vi "Generate Tree Data Representation.vi"(8 "error in (no error)":errorcluster, 11 "ParseGDSII in":refnum<class "ParseGDSII.lvclass">) -> (0 "error out":errorcluster, 3 "ParseGDSII out":refnum<class "ParseGDSII.lvclass">)   [LabVIEW 2019, in "ParseGDSII.lvclass"]
uses:
  ParseGDSII.lvclass
  ParseGDSII.lvclass/ParseGDSII.ctl
  Fast Tree/Fast Tree.lvclass
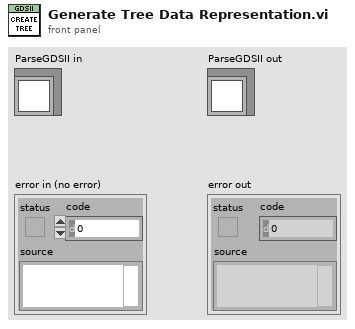
[diagram p1: front panel]
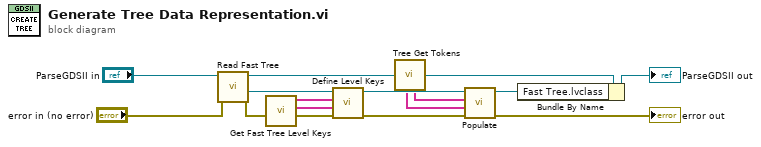
[diagram p0: block diagram]
diagram:
  n1 = call "Read Fast Tree.vi"("error in"="error in (no error)", "ParseGDSII in"="ParseGDSII in") -> ("error out"=w5:errorcluster, "Fast Tree.lvclass"=w4:refnum<class "Fast Tree.lvclass">, "ParseGDSII out"=w3:refnum<class "ParseGDSII.lvclass">)  [unwired: 6 in, 1 out]
  n2 = call "Get Fast Tree Level Keys.vi"("error in (no error)"=w5) -> ("error out"=w11:errorcluster, "Level Down Keys"=w9:string[], "Level Up Keys"=w10:string[])  [unwired: 8 in]
  n3 = call "Define Level Keys.vi"("error in"=w11, "Level Down Keys"=w9, "Level Up Keys"=w10, "Fast Tree in"=w4) -> ("error out"=w15:errorcluster, "Fast Tree out"=w13:refnum<class "Fast Tree.lvclass">)  [unwired: 6 in]
  n4 = call "Tree Get Tokens.vi"("ParseGDSII in"=w3) -> ("Record Payloads"=w2:string[], "Record Types"=w1:string[], "ParseGDSII out"=w8:refnum<class "ParseGDSII.lvclass">)
  n5 = call "Populate.vi"("error in"=w15, "Values In"=w2, "Keys In"=w1, "Fast Tree in"=w13) -> ("error out"=→"error out":errorcluster, "Fast Tree out"=w14:refnum<class "Fast Tree.lvclass">)  [unwired: 5 in, 1 out]
  n6 = Bundle By Name(cluster=w8, "Fast Tree.lvclass"=w14) -> (→"ParseGDSII out":refnum<class "ParseGDSII.lvclass">)
